vi "ActionVIOnCompile.vi"(8 "error in":errorcluster, 11 "Device Item Ref in":T1 format="%.0x") -> (0 "error out":errorcluster)   [LabVIEW 2020, in "Ballard ARINC 429 System Explorer.lvlib"]
uses:
  Ballard ARINC 429 System Explorer.lvlib
  <vilib>/NI VeriStand/Custom Device API/Custom Device Item Ref.ctl
  Includes/Ballard ARINC 429 Engine.lvlibp/Engine/Interfaces/Execution Unit Factory/Execution Unit Factory.lvclass
  Includes/Ballard ARINC 429 Engine.lvlibp/Engine/Implementation/Execution Unit Factory/Execution Unit Factory.lvclass
  C:/dev/git/niveristand-ballard-arinc429-custom-device/Includes/Ballard ARINC 429 Engine.lvlibp/Engine/Interfaces/Execution Unit Factory/Execution Unit Factory.lvclass
  Includes/Ballard ARINC 429 Engine.lvlibp/Engine/Implementation/Shared Resources Factory/Shared Resources Factory.lvclass
  C:/dev/git/niveristand-ballard-arinc429-custom-device/Includes/Ballard ARINC 429 Engine.lvlibp/Engine/Interfaces/Shared Resources Factory/Shared Resources Factory.lvclass
  Includes/Ballard ARINC 429 Engine.lvlibp/Engine/Interfaces/Shared Resources Factory/Shared Resources Factory.lvclass
  Includes/Ballard ARINC 429 Engine.lvlibp/Engine/Custom Device/Compiled.Settings.ctl
  Includes/Ballard ARINC 429 Engine.lvlibp/Engine/Custom Device/Inline Execution Unit Compiled Information.ctl
  Includes/Ballard ARINC 429 Engine.lvlibp/1abvi3w/vi.lib/NI VeriStand/Custom Device API/Data Reference.ctl
  Includes/Ballard ARINC 429 Engine.lvlibp/1abvi3w/vi.lib/NI VeriStand/Custom Device API/Block Data Reference.ctl
  Includes/Ballard ARINC 429 Engine.lvlibp/Engine/Custom Device/Asynchronous Execution Unit Compiled Information.ctl
  Shared/Constants.vi
  <vilib>/NI VeriStand/Custom Device API/Set Item Property (Variant).vi
  <vilib>/NI VeriStand/Custom Device API/Custom Device API.lvlib
  Includes/Ballard ARINC 429 Engine.lvlibp/1abvi3w/vi.lib/NI VeriStand/Custom Device API/Custom Device API.lvlib
  Includes/Ballard ARINC 429 Engine.lvlibp/Engine/Custom Device/Custom Device.lvlib
  Shared/Ballard ARINC 429 Shared.lvlib
  Includes/Ballard ARINC 429 System Explorer.lvlibp/System Explorer/Implementation/Implementation.lvlib
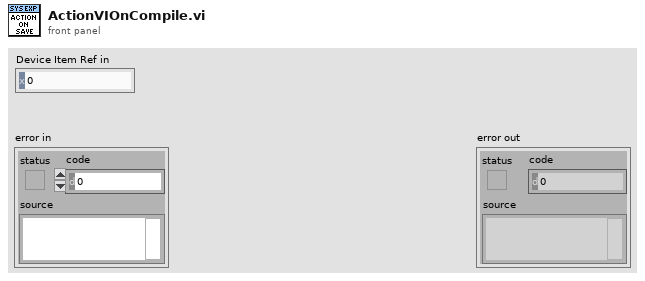
[diagram p1: front panel]
types:
  T1 = typedef "Custom Device API.lvlib/Custom Device Item Ref.ctl" = u64
  T2 = typedef "Ballard ARINC 429 System Explorer.lvlibp/Custom Device API.lvlib/Custom Device Item Ref.ctl" = u64
  T3 = typedef "Ballard ARINC 429 Engine.lvlibp/Custom Device.lvlib/Compiled.Settings.ctl" = cluster{"Name":string, "Inline Execution Unit Compiled Information":T4[], "Asynchronous Execution Unit Compiled Information":T7[], "flattened shared resources":string}
  T4 = typedef "Ballard ARINC 429 Engine.lvlibp/Custom Device.lvlib/Inline Execution Unit Compiled Information.ctl" = cluster{"Flattened Execution Unit":string, "Incoming Buffer":dbl[], "Outgoing Buffer":dbl[], "Incoming Data References":T5[], "Outgoing Data References":T6[]}
  T5 = typedef "Ballard ARINC 429 Engine.lvlibp/Custom Device API.lvlib/Data Reference.ctl" = i32
  T6 = typedef "Ballard ARINC 429 Engine.lvlibp/Custom Device API.lvlib/Block Data Reference.ctl" = cluster{"Data Reference":T5, "Offset":u64, "Length":u64}
  T7 = typedef "Ballard ARINC 429 Engine.lvlibp/Custom Device.lvlib/Asynchronous Execution Unit Compiled Information.ctl" = cluster{"Flattened Execution Unit":string, "Incoming Channel Group Name":string, "Outgoing Channel Group Name":string, "ReadWrite Channel Group Name":string}
  T8 = typedef "Custom Device API.lvlib/Custom Device Item Info.ctl" = cluster{"Name":string, "Is Channel":bool, "GUID":string, "Is Waveform":bool}
  T9 = typedef "Ballard ARINC 429 Engine.lvlibp/Interfaces.lvlib/Execution Unit Information.ctl" = cluster{"Execution Unit":refnum<class "Execution Unit.lvclass">, "Incoming Channels":T10[], "Outgoing Channels":T10[], "ReadWrite Channels":T10[]}
  T10 = typedef "Ballard ARINC 429 Engine.lvlibp/Custom Device API.lvlib/Custom Device Item Ref.ctl" = u64
  T11 = typedef "Ballard ARINC 429 Shared.lvlib/Inline Execution Unit Compiled Information.ctl" = cluster{"Flattened Execution Unit":string, "Incoming Buffer":dbl[], "Outgoing Buffer":dbl[], "Incoming Data References":T12[], "Outgoing Data References":T13[]}
  T12 = typedef "Custom Device API.lvlib/Data Reference.ctl" = i32
  T13 = typedef "Custom Device API.lvlib/Block Data Reference.ctl" = cluster{"Data Reference":T12, "Offset":u64, "Length":u64}
  T14 = typedef "Ballard ARINC 429 Shared.lvlib/Asynchronous Execution Unit Compiled Information.ctl" = cluster{"Flattened Execution Unit":string, "Incoming Channel Group Name":string, "Outgoing Channel Group Name":string, "ReadWrite Channel Group Name":string}
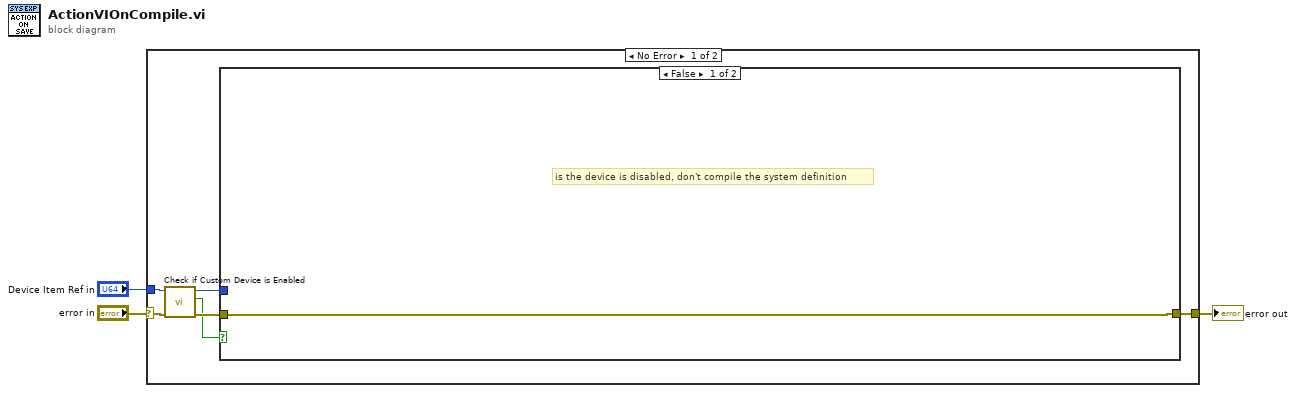
[diagram p0: block diagram]
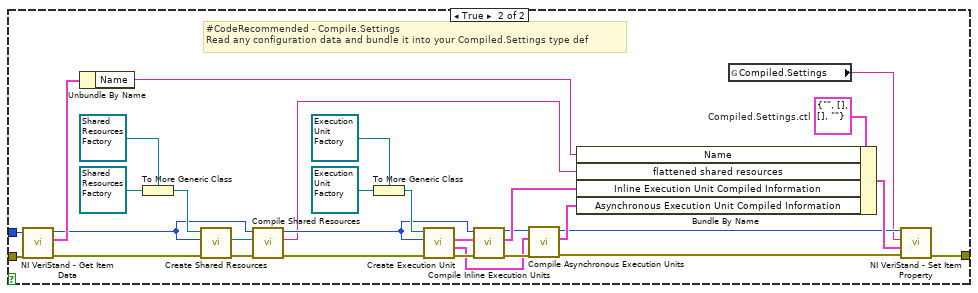
[diagram p2: hidden frame]
diagram:
  n1 = case shown="No Error" "error in" {
    selector: "error in" -> [w4 w41]
    tunnel: [w9 w41] -> w2
    tunnel: "Device Item Ref in" -> [w5 _]
    frame No Error {
      n2 = call "Check if Custom Device is Enabled.vi"("error in (no error)"=w4, "Ballard ARINC 429 ref"=w5) -> ("error out"=w7:errorcluster, "Custom Device is Enabled"=w6:bool, "Ballard ARINC 429 ref"=w8:T2)  [unwired: 7 in]
      n3 = case shown="False" w6 {
        tunnel: [w10 w39] -> w9
        tunnel: w7 -> [w10 w12]
        tunnel: w8 -> [_ w11]
        frame False {
          # "is the device is disabled, don't compile the system definition"
        }
        frame True {
          w14 = T3 {"Name"="", "Inline Execution Unit Compiled Information"=[], "Asynchronous Execution Unit Compiled Information"=[], "flattened shared resources"=""}  # Compiled.Settings.ctl
          # "#CodeRecommended - Compile.Settings\nRead any configuration data and bundle it into your Compiled.Settings type def"
          n4 = call <vilib>:"NI VeriStand - Get Item Data.vi"("error in (no error)"=w12, "Item Ref in"=w11) -> ("error out"=w24:errorcluster, "Item Info"=w38:T8, "Item Ref out"=w20:T1)  [unwired: 6 in, 1 out]
          n5 = Unbundle By Name(w38) -> ("Name"=w36:string)
          n6 = To More Generic Class(target class=refnum<class "Shared Resources Factory.lvclass"> refnum ("Communication Bus Template Interfaces:Interfaces.lvlib:Shared Resources Factory.lvclass"), reference=refnum<class "Shared Resources Factory.lvclass"> refnum ("Shared Resources Factory in")) -> (generic class reference=w21:refnum<class "Shared Resources Factory.lvclass">)
          n7 = call-dynamic "Create Shared Resources.vi"("error in"=w24, "custom device ref"=w20, "shared resources factory in"=w21) -> ("error out"=w19:errorcluster, "shared resources"=w16:refnum<class "Shared Resources.lvclass">)  [unwired: 6 in, 1 out]
          n8 = call "Compile Shared Resources.vi"("error in"=w19, "shared resources"=w16, "device ref in"=w20) -> ("error out"=w18:errorcluster, "flattened shared resources"=w15:string, "device ref out"=w17:T1)  [unwired: 6 in]
          n9 = To More Generic Class(target class=refnum<class "Execution Unit Factory.lvclass"> refnum ("Communication Bus Template Interfaces:Interfaces.lvlib:Execution Unit Factory.lvclass"), reference=refnum<class "Execution Unit Factory.lvclass"> refnum ("Communication Bus Template Interfaces:Implementation.lvlib:Execution Unit Factory.lvclass")) -> (generic class reference=w35:refnum<class "Execution Unit Factory.lvclass">)
          n10 = call-dynamic "Create Execution Unit.vi"("error in"=w18, "Item Ref"=w17, "Execution Unit Factory in"=w35) -> ("error out"=w37:errorcluster, "Asynchronous Execution Units"=w27:T9[], "Inline Execution Units"=w33:T9[])  [unwired: 5 in, 1 out]
          n11 = call "Compile Inline Execution Units.vi"("error in"=w37, "Inline Execution Units"=w33, "Device Ref in"=w17) -> ("error out"=w32:errorcluster, "Compiled Inline Execution Units"=w34:T11[], "Device Ref out"=w31:T1)  [unwired: 6 in]
          n12 = call "Compile Asynchronous Execution Units.vi"("Device Ref in"=w31, "Asynchronous Execution Units"=w27, "error in"=w32) -> ("Device Ref out"=w28:T1, "Compiled Asynchronous Execution Units"=w30:T14[], "error out"=w29:errorcluster)  [unwired: 5 in]
          n13 = Bundle By Name(cluster=w14, "Name"=w36, "flattened shared resources"=w15, "Inline Execution Unit Compiled Information"=w34, "Asynchronous Execution Unit Compiled Information"=w30) -> (w40:T3)
          n14 = global read "Constants.vi" "Compiled.Settings"() -> (w13:string)
          n15 = call-poly <vilib>:"NI VeriStand - Set Item Property.vi"("error in (no error)"=w29, "Value"=w40, "Property Name"=w13, "Item Ref in"=w28) -> ("error out"=w39:errorcluster)  [unwired: 5 in, 2 out]
        }
      }
    }
    frame Error {
    }
  }
  "error out" <- w2
